vi "Test surveillance reg.vi"() -> ()   [LabVIEW 2022 SP3]
uses:
  Enum/Enum r16.ctl
  Variables globales/Variable glob generale.vi
panel:
  in  "annuler":bool
  in  "Bouton OK":bool
  in  "Mot de passe (admin station) :":string
  # "test surveillance régulateurs"
  # "La surveillance compare les alarmes envoyées aux régulateurs (et mémorisées par le logiciel de gestion des régulateurs) avec celles qui sont dans les régulateurs.\n\nPour simplifier le test, ce sont les alarmes mémorisées par le logiciel qui seront changées avant comparaison."
  # "CE TEST DOIT :\n- ARRETER LA REGULATION EN COURS\n- CHANGER LES VALEURS DES ALARMES DU REGULATEUR\n- METTRE LA CONSIGNE LOCALE  A LA VALEUR DE LA MESURE ACTUELLE"
  # "Ce logiciel et les informations qu'il contient, sont la propriété de l’IAS et ne peuvent être diffusés sans l’autorisation de la Station d’étalonnage"
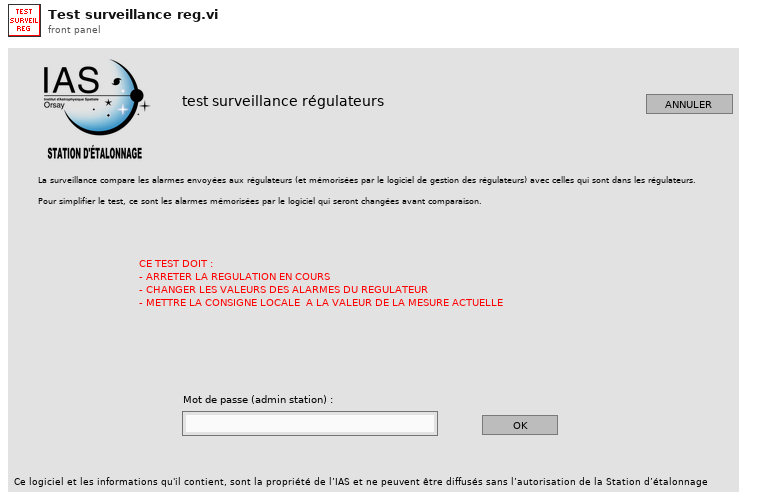
[diagram p1: front panel]
types:
  T1 = typedef "Enum r16.ctl" = enum16{"init", "attente", "comparaison", "modif al", "sortie"}
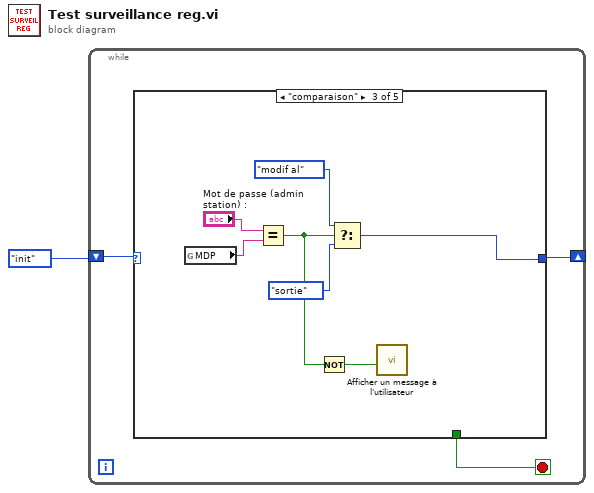
[diagram p0: block diagram]
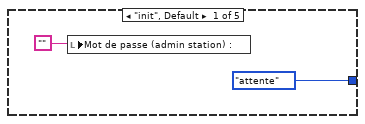
[diagram p2: hidden frame]
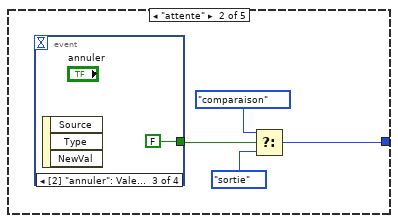
[diagram p3: hidden frame]
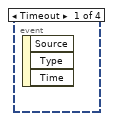
[diagram p4: hidden frame]
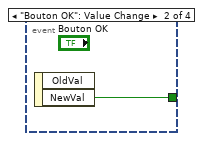
[diagram p5: hidden frame]
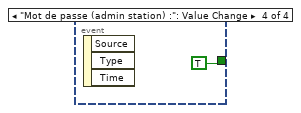
[diagram p6: hidden frame]
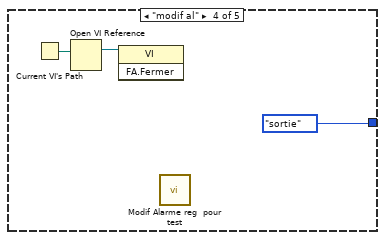
[diagram p7: hidden frame]
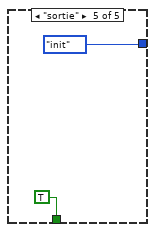
[diagram p8: hidden frame]
diagram:
  n1 = while {
    shift-right: [w3] -> _
    shift-left: Enum_r16."init" ("Énum") -> [w4]
    stop <- w2 stop-if-true
    n2 = case shown="\"comparaison\"" w4 {
      tunnel: [Enum_r16."attente" ("Énum") w7 w16 Enum_r16."sortie" ("Énum") Enum_r16."init" ("Énum")] -> w3
      tunnel: [_ _ _ _ TRUE] -> w2
      frame "init", Default {
        n3 = local write "Mot de passe (admin station) :"("") -> ()
      }
      frame "attente" {
        n4 = event shown="[2] \"annuler\": Valeur changée" {
          selector: _ -> [_ _ _ _]
          dyn-events: _ -> [_ _ _ _]
          timeout: _ -> [_ _ _ _]
          tunnel: [_ w11 FALSE TRUE] -> w10
          event Timeout {
            n5 = event-data() -> ()  [unwired: 1 in, 3 out]
          }
          event "Bouton OK": Value Change {
            n6 = event-data() -> ("NewVal"=w11:bool)  [unwired: 1 in, 1 out]
          }
          event "annuler": Value Change {
            n7 = event-data() -> ()  [unwired: 1 in, 3 out]
          }
          event "Mot de passe (admin station) :": Value Change {
            n8 = event-data() -> ()  [unwired: 1 in, 3 out]
          }
        }
        n9 = Select(t=Enum_r16."comparaison" ("Énum"), s=w10, f=Enum_r16."sortie" ("Énum")) -> (s? t:f=w7:T1)
      }
      frame "comparaison" {
        n10 = global read "Variable glob generale.vi" "MDP"() -> (w20:string)
        n11 = Equal?(x="Mot de passe (admin station) :", y=w20) -> (x = y?=w15:bool)
        n12 = Not(x=w15) -> (.not. x?=w14:bool)
        n13 = Select(t=Enum_r16."modif al" ("Énum"), s=w15, f=Enum_r16."sortie" ("Énum")) -> (s? t:f=w16:T1)
        n14 = call "Afficher un message à l'utilisateur"("Enable"=w14) -> ()  [unwired: 9 in, 2 out]
      }
      frame "modif al" {
        n15 = Current VI's Path() -> (path=w22:path)
        n16 = Open VI Reference(vi path=w22) -> (vi reference=w21:refnum<vi>)  [unwired: 5 in, 1 out]
        n17 = invoke class="VI" method="FA.Fermer"(reference=w21) -> ()  [unwired: 2 in, 3 out]
        n18 = call "Modif Alarme reg  pour test.vi"() -> ()  [unwired: 12 in]
      }
      frame "sortie" {
      }
    }
  }
